vi "Popup_Begin.vi"(8 "error in (no error)":errorcluster={"status"=FALSE, "code"=0, "source"="\"\""}, 10 "request ID":string, 11 "Popup definition":string) -> (0 "error out":errorcluster={"status"=FALSE, "code"=0, "source"="\"\""}, 2 "status ok":bool, 3 "Popup session state":string)   [LabVIEW 2026]
doc: "INTENT: Request an operator or feedback acknowledgement. LOGIC: Post prompt event to Host; register independent feedback and elapsed requirements."
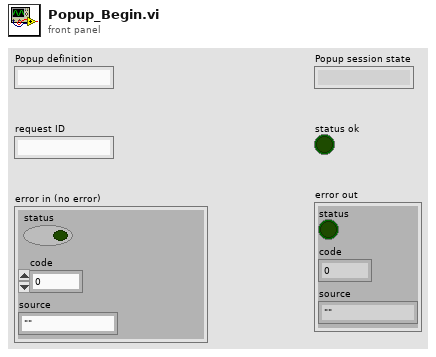
[diagram p1: front panel]
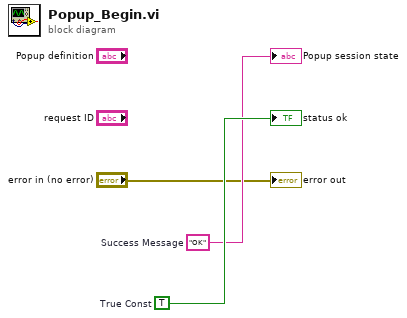
[diagram p0: block diagram]
diagram:
  w3 = TRUE  # True Const
  w2 = "OK"  # Success Message
  "Popup session state" <- w2
  "status ok" <- w3
  "error out" <- "error in (no error)"
